vi "DiffDrivePoseEst2_AddVisionMeasurement.vi"(9 "TImeStamp_Seconds":dbl=0.02, 10 "visionRobotPose":T6={"TRANSLATION"={"X"=0.0, "Y"=0.0}, "ROTATION"={"VALUE"=0.0, "COS"=1.0, "SIN"=0.0}} {"ROTATION"."SIN" format="%13.4f"; "ROTATION"."COS" format="%13.4f"; "ROTATION"."VALUE" format="%13.4f"; "TRANSLATION"."Y" format="%14.3f"; "TRANSLATION"."X" format="%14.3f"}, 11 "in DiffDrivePoseEst2":T1={"M_Vision_K"=[], "m_nominal_dT"=0.0, "m_PrevTime_Sec"=0.0, "Pose_Buffer"={"TimeStamps"=[], "DataArray"=[], "Min_TimeStamp"=0.0, "Max_TimeStamp"=0.0, "ItemCount"=0, "MaxBufferTime"=0.0}, "Diff_Drive_Kinematics"={"TrackWidth_Meters"=0.0}, "Diff_Drive_Odom_2"={"M_POSE_Meters"={"TRANSLATION"={"X"=0.0, "Y"=0.0}, "ROTATION"={"VALUE"=0.0, "COS"=1.0, "SIN"=0.0}}, "M_GyroOffset"={"VALUE"=0.0, "COS"=1.0, "SIN"=0.0}, "M_PrevAngle"={"VALUE"=0.0, "COS"=1.0, "SIN"=0.0}, "M_PrevLeftDist_M"=0.0, "M_PrevRightDist_M"=0.0, "M_InitLeftDist_M"=0.0, "M_InitRightDist_M"=0.0}, "M_Q"=[[0.0], [0.0], [0.0]]} {"Diff_Drive_Odom_2"."M_PrevAngle"."SIN" format="%13.4f"; "Diff_Drive_Odom_2"."M_PrevAngle"."COS" format="%13.4f"; "Diff_Drive_Odom_2"."M_PrevAngle"."VALUE" format="%13.4f"; "Diff_Drive_Odom_2"."M_GyroOffset"."SIN" format="%13.4f"; "Diff_Drive_Odom_2"."M_GyroOffset"."COS" format="%13.4f"; "Diff_Drive_Odom_2"."M_GyroOffset"."VALUE" format="%13.4f"; "Diff_Drive_Odom_2"."M_POSE_Meters"."ROTATION"."SIN" format="%13.4f"; "Diff_Drive_Odom_2"."M_POSE_Meters"."ROTATION"."COS" format="%13.4f"; "Diff_Drive_Odom_2"."M_POSE_Meters"."ROTATION"."VALUE" format="%13.4f"; "Diff_Drive_Odom_2"."M_POSE_Meters"."TRANSLATION"."Y" format="%14.3f"; "Diff_Drive_Odom_2"."M_POSE_Meters"."TRANSLATION"."X" format="%14.3f"; "Diff_Drive_Kinematics"."TrackWidth_Meters" format="%20.4f"}) -> (0 "Error":bool, 3 "Out DiffDrivePoseEst2":T1={"M_Vision_K"=[], "m_nominal_dT"=0.0, "m_PrevTime_Sec"=0.0, "Pose_Buffer"={"TimeStamps"=[], "DataArray"=[], "Min_TimeStamp"=0.0, "Max_TimeStamp"=0.0, "ItemCount"=0, "MaxBufferTime"=0.0}, "Diff_Drive_Kinematics"={"TrackWidth_Meters"=0.0}, "Diff_Drive_Odom_2"={"M_POSE_Meters"={"TRANSLATION"={"X"=0.0, "Y"=0.0}, "ROTATION"={"VALUE"=0.0, "COS"=1.0, "SIN"=0.0}}, "M_GyroOffset"={"VALUE"=0.0, "COS"=1.0, "SIN"=0.0}, "M_PrevAngle"={"VALUE"=0.0, "COS"=1.0, "SIN"=0.0}, "M_PrevLeftDist_M"=0.0, "M_PrevRightDist_M"=0.0, "M_InitLeftDist_M"=0.0, "M_InitRightDist_M"=0.0}, "M_Q"=[[0.0], [0.0], [0.0]]} {"Diff_Drive_Odom_2"."M_PrevAngle"."SIN" format="%13.4f"; "Diff_Drive_Odom_2"."M_PrevAngle"."COS" format="%13.4f"; "Diff_Drive_Odom_2"."M_PrevAngle"."VALUE" format="%13.4f"; "Diff_Drive_Odom_2"."M_GyroOffset"."SIN" format="%13.4f"; "Diff_Drive_Odom_2"."M_GyroOffset"."COS" format="%13.4f"; "Diff_Drive_Odom_2"."M_GyroOffset"."VALUE" format="%13.4f"; "Diff_Drive_Odom_2"."M_POSE_Meters"."ROTATION"."SIN" format="%13.4f"; "Diff_Drive_Odom_2"."M_POSE_Meters"."ROTATION"."COS" format="%13.4f"; "Diff_Drive_Odom_2"."M_POSE_Meters"."ROTATION"."VALUE" format="%13.4f"; "Diff_Drive_Odom_2"."M_POSE_Meters"."TRANSLATION"."Y" format="%14.3f"; "Diff_Drive_Odom_2"."M_POSE_Meters"."TRANSLATION"."X" format="%14.3f"; "Diff_Drive_Kinematics"."TrackWidth_Meters" format="%20.4f"})   [LabVIEW 2019, in "Trajectory_Library.lvlib"]
doc: "Add a vision measurement to the Unscented Kalman Filter. This will correct the odometry pose estimate while still accounting for measurement noise.\n \nThis method can be called as infrequently as you want, as long as you are calling DifferentialDrivePoseEstimator_update every loop.\n\nTo promote stability of the pose estimate and make it robust to bad vision data, we recommend only adding vision measurements that are already within one meter or so of the current pose estimate.\n\n Inputs:\n - InDIffDrivePoseEstimate -- Data cluster for this system\n - visionRobotPoseMeters -- The pose of the robot as measured by the vision camera.\n - timestampSeconds -- The timestamp of the vision measurement in seconds. Note that if you don't use your own time source by calling DifferentialDrivePoseEstimator_updateWithTime then you must use a timestamp with an epoch since FPGA startup (i.e. the epoch of this timestamp is the same epoch as Timer.getFPGATimestamp.) This means that you should use Timer.getFPGATimestamp as your time source in this case.\n\nOutputs:\n - OutDIffDrivePoseEstimate -- Data cluster for this system\n - Error -- Returns TRUE if an error occured."
uses:
  Trajectory_Library.lvlib
  TypeDef/DIFF_DRIVE_POSE_EST2.ctl
  <vilib>/Analysis/Matrix/Datatypes/RealMatrix.ctl
  TypeDef/TIME_INTERPOLATABLE_VARIANT.ctl
  TypeDef/DIFF_DRIVE_KINEMATICS.ctl
  TypeDef/DIFF_DRIVE_ODOM2.ctl
  TypeDef/POSE2D.ctl
  TypeDef/TRANSLATION2D.ctl
  TypeDef/ROTATION2D.ctl
  <vilib>/Analysis/baseanly.llb/Real A x B.vi
  MatBuilder_Create.vi
  Pose2d_getRotation.vi
  Rotation2d_Minus.vi
  TimeInterpVariant_CleanUp.vi
  Rotation2d_UnaryMinus.vi
  Rotation2d_RotateBy.vi
  Rotation2d_CreateAngle.vi
  Rotation2d_CreateXY.vi
  Util_CalcDist.vi
  <vilib>/gmath/interp.llb/Search Ordered Table.vi
  DiffDrivePoseEst2_InterpRecord_Interp.vi
  <vilib>/Analysis/NI_AALBase.lvlib
  <vilib>/Analysis/Matrix/NI_Matrix.lvlib
panel:
  # "NOT A PARAMETER, JUST A DATA TYPE"
  # "<3, 1>"
  # "<3, 3>"
  # "<3, 1>"
  # "<3, 3>"
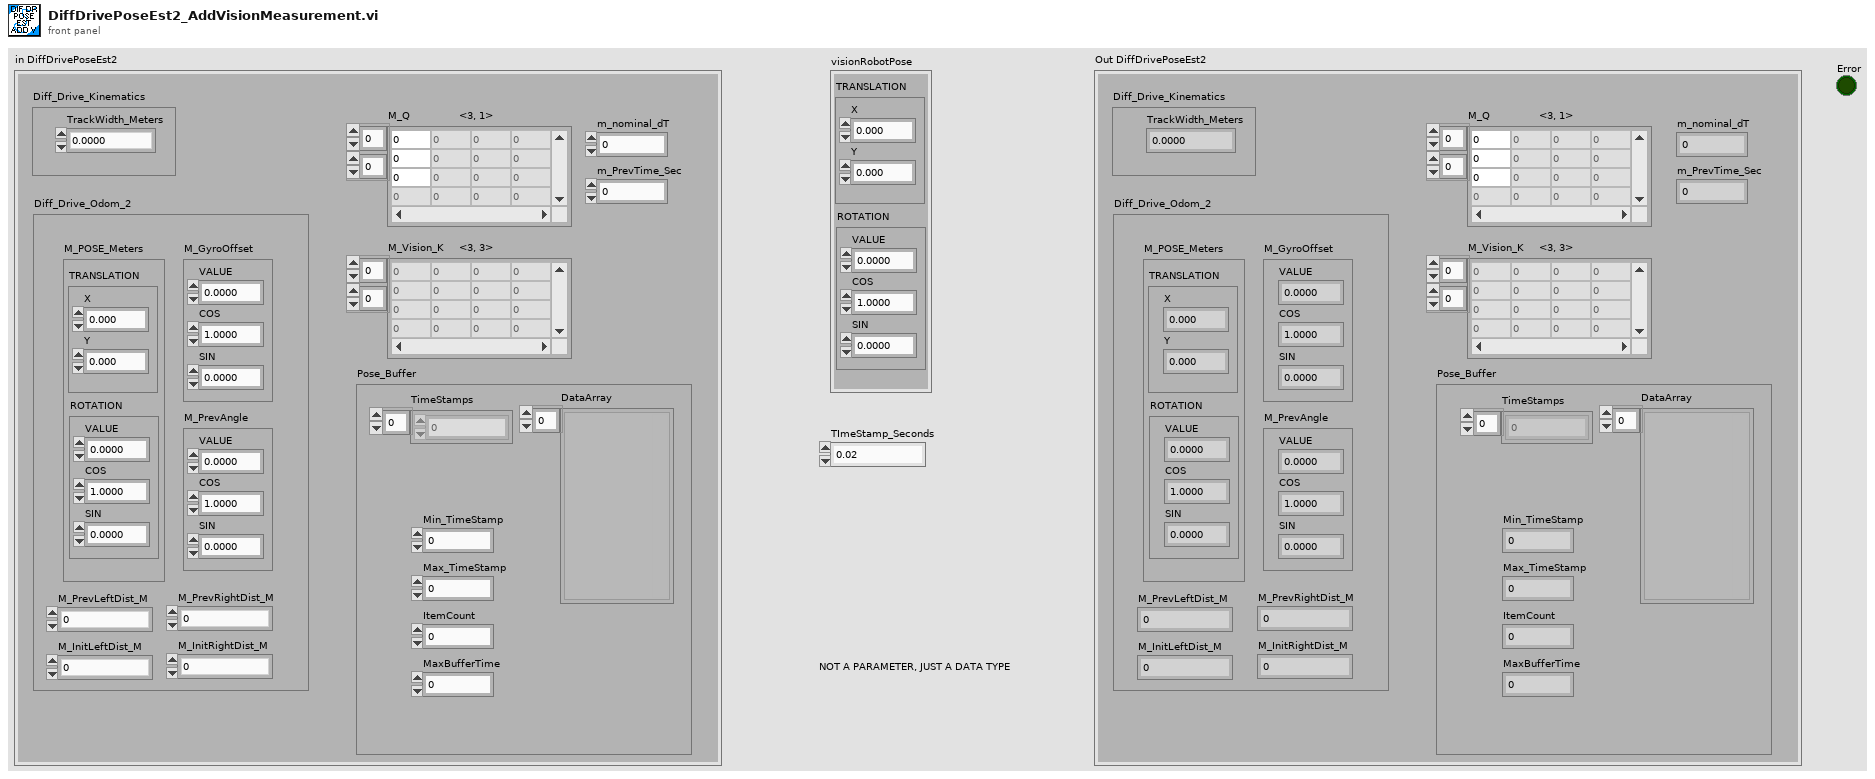
[diagram p1: front panel]
types:
  T1 = typedef "Trajectory_Library.lvlib/DIFF_DRIVE_POSE_EST2.ctl" = cluster{"M_Vision_K":T2, "m_nominal_dT":dbl, "m_PrevTime_Sec":dbl, "Pose_Buffer":T3, "Diff_Drive_Kinematics":T4, "Diff_Drive_Odom_2":T5, "M_Q":T2}
  T2 = typedef "NI_Matrix.lvlib/RealMatrix.ctl" = dbl[][]
  T3 = typedef "Trajectory_Library.lvlib/TIME_INTERPOLATABLE_VARIANT.ctl" = cluster{"TimeStamps":dbl[], "DataArray":variant[], "Min_TimeStamp":dbl, "Max_TimeStamp":dbl, "ItemCount":i32, "MaxBufferTime":dbl}
  T4 = typedef "Trajectory_Library.lvlib/DIFF_DRIVE_KINEMATICS.ctl" = cluster{"TrackWidth_Meters":dbl}
  T5 = typedef "Trajectory_Library.lvlib/DIFF_DRIVE_ODOM2.ctl" = cluster{"M_POSE_Meters":T6, "M_GyroOffset":T8, "M_PrevAngle":T8, "M_PrevLeftDist_M":dbl, "M_PrevRightDist_M":dbl, "M_InitLeftDist_M":dbl, "M_InitRightDist_M":dbl}
  T6 = typedef "Trajectory_Library.lvlib/POSE2D.ctl" = cluster{"TRANSLATION":T7, "ROTATION":T8}
  T7 = typedef "Trajectory_Library.lvlib/TRANSLATION2D.ctl" = cluster{"X":dbl, "Y":dbl}
  T8 = typedef "Trajectory_Library.lvlib/ROTATION2D.ctl" = cluster{"VALUE":dbl, "COS":dbl, "SIN":dbl}
  T9 = typedef "Trajectory_Library.lvlib/DIFF_DRIVE_POSE_EST2_INTERP_RECORD.ctl" = cluster{"PoseMeters":T6, "GyroAngle":T8, "LeftMeters":dbl, "RightMeters":dbl}
  T10 = typedef "Trajectory_Library.lvlib/TWIST2D.ctl" = cluster{"dX":dbl, "dY":dbl, "dTHETA":dbl}
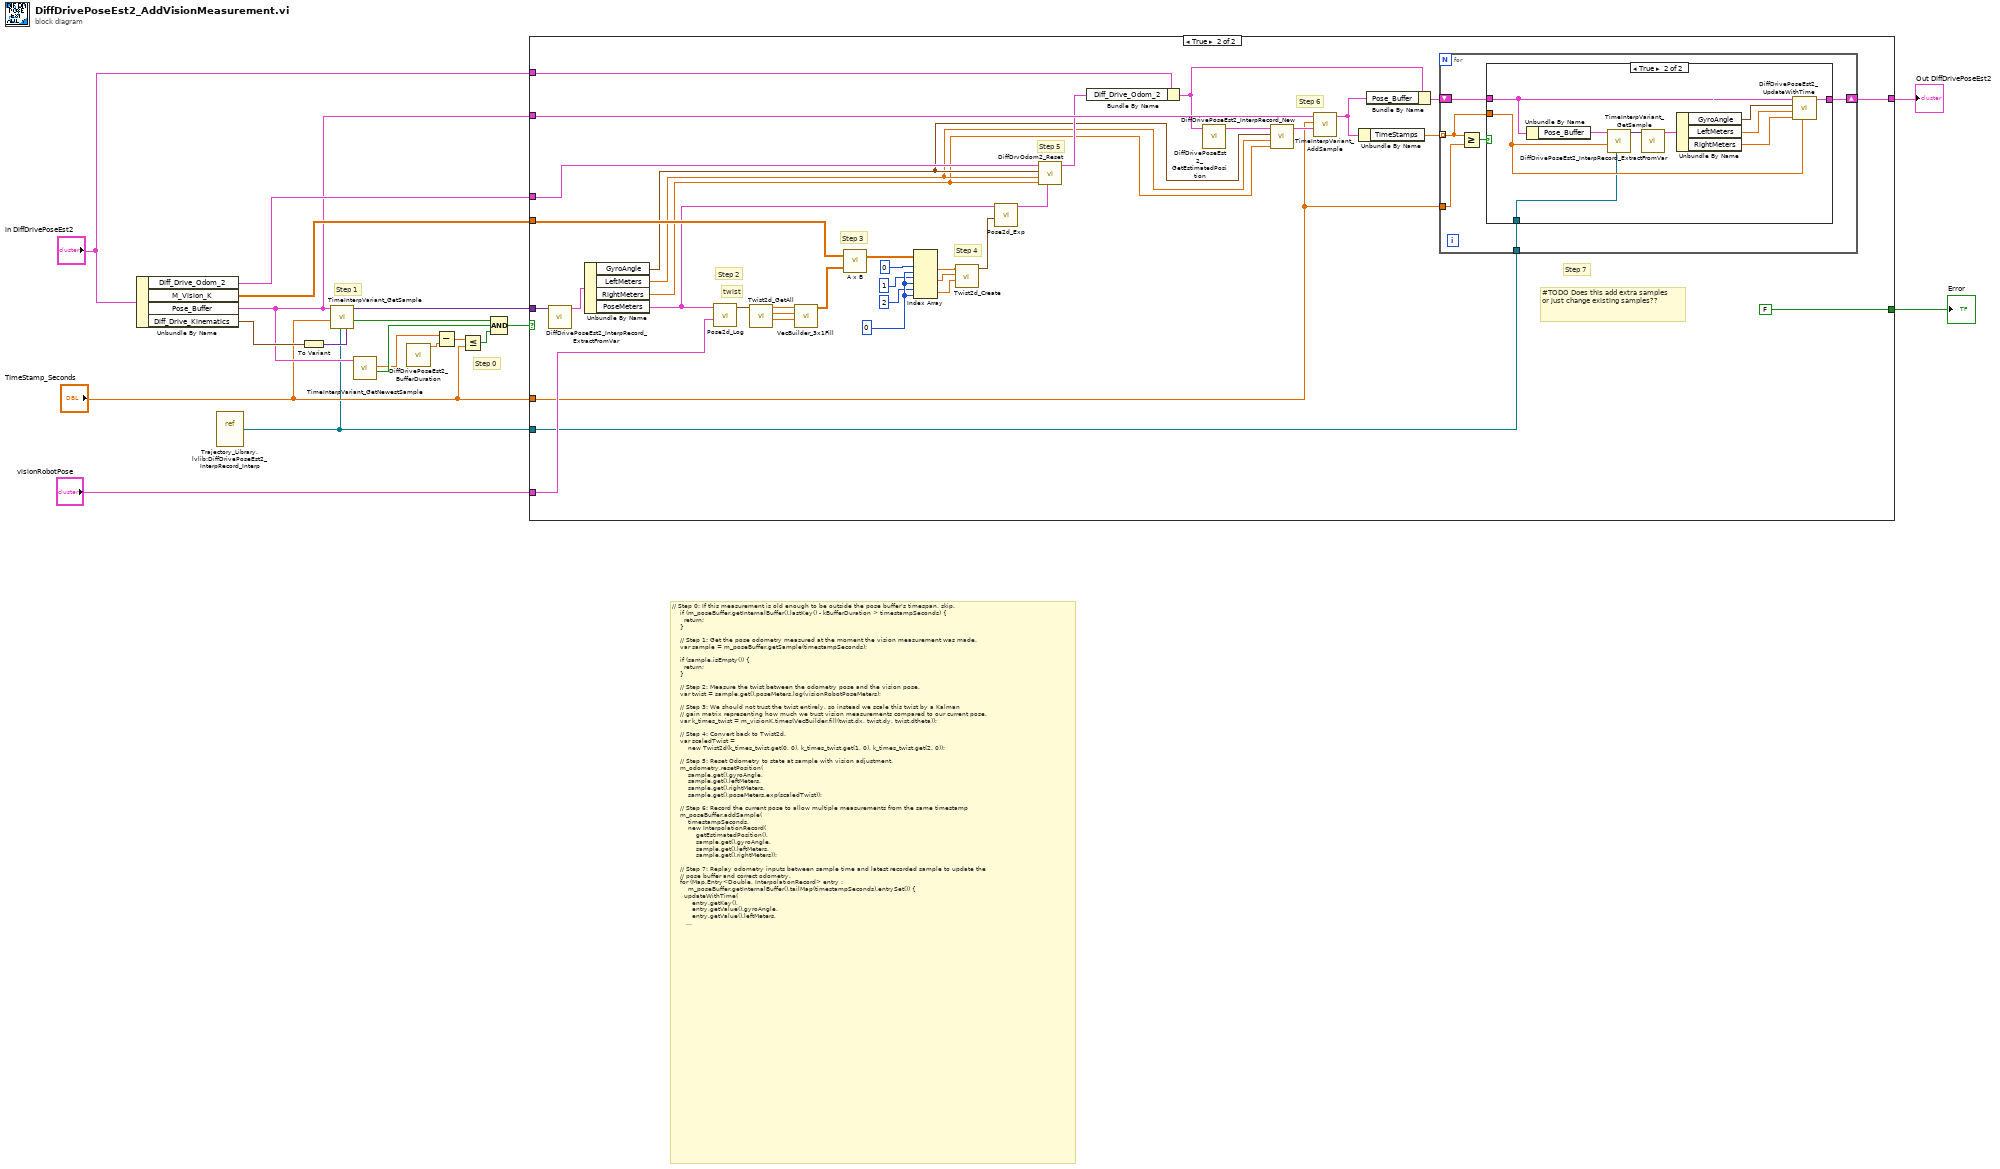
[diagram p0: block diagram]
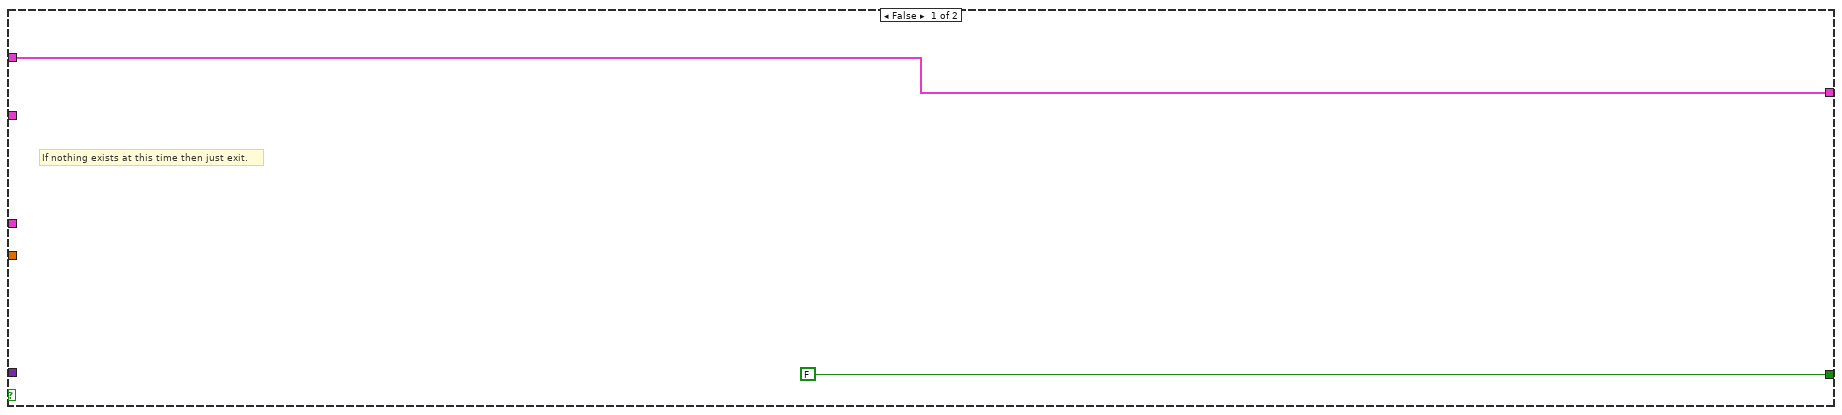
[diagram p2: hidden frame]
diagram:
  # "Step 0"
  # "Step 1"
  # "// Step 0: If this measurement is old enough to be outside the pose buffer's timespan, skip.\n    if (m_poseBuffer.getInternalBuffer().lastKey() - kBufferDuration > timestampSeconds) {\n      return;\n    }\n\n    // Step 1: Get the pose odometry measured at the moment the vision measurement was made.\n    var sample = m_poseBuffer.getSample(timestampSeconds);\n\n    if (sample.isEmpty()) {\n      return;\n    }\n\n    // Step 2: Measure the twist between the odometry pose and the vision pose.\n    var twist = sample.get().poseMeters.log(visionRobotPoseMeters);\n\n    // Step 3: We should not trust the twist entirely, so instead we scale this twist by a Kalman\n    // gain matrix representing how much we trust vision measurements compared to our current pose.\n    var k_times_twist = m_visionK.times(VecBuilder.fill(twist.dx, twist.dy, twist.dtheta));\n\n    // Step 4: Convert back to Twist2d.\n    var scaledTwist =\n        new Twist2d(k_times_twist.get(0, 0), k_times_twist.get(1, 0), k_times_twist.get(2, 0));\n\n    // Step 5: Reset Odometry to state at sample with vision adjustment.\n    m_odometry.resetPosition(\n        sample.get().gyroAngle,\n        sample.get().leftMeters,\n        sample.get().rightMeters,\n        sample.get().poseMeters.exp(scaledTwist));\n\n    // Step 6: Record the current pose to allow multiple measurements from the same timestamp\n    m_poseBuffer.addSample(\n        timestampSeconds,\n        new InterpolationRecord(\n            getEstimatedPosition(),\n            sample.get().gyroAngle,\n            sample.get().leftMeters,\n            sample.get().rightMeters));\n\n    // Step 7: Replay odometry inputs between sample time and latest recorded sample to update the\n    // pose buffer and correct odometry.\n    for (Map.Entry<Double, InterpolationRecord> entry :\n        m_poseBuffer.getInternalBuffer().tailMap(timestampSeconds).entrySet()) {\n      updateWithTime(\n          entry.getKey(),\n          entry.getValue().gyroAngle,\n          entry.getValue().leftMeters,\n          entry.getValue().rightMeters);\n    }"
  n1 = Unbundle By Name("in DiffDrivePoseEst2") -> ("Diff_Drive_Odom_2"=w11:T5, "M_Vision_K"=w12:T2, "Pose_Buffer"=w10:T3, "Diff_Drive_Kinematics"=w14:T4)
  n2 = vi-ref "Trajectory_Library.lvlib:DiffDrivePoseEst2_InterpRecord_Interp.vi"() -> (w1:refnum<vi>)
  n3 = To Variant(anything=w14) -> (Variant=w15:variant)
  n4 = call "TimeInterpVariant_GetSample.vi"("Extra"=w15, "Interpolate\nReference"=w1, "TimeStamp"="TImeStamp_Seconds", "TimeInterpVariant"=w10) -> ("IsPresent"=w9:bool, "OutputVariant"=w13:variant)  [unwired: 6 in]
  n5 = call "TimeInterpVariant_GetNewestSample.vi"("TimeInterpVariant"=w10) -> ("IsPresent"=w8:bool, "TimeStamp"=w7:dbl)  [unwired: 8 in, 1 out]
  n6 = call "DiffDrivePoseEst2_BufferDuration.vi"() -> ("Buffer Duration (Sec)"=w3:dbl)  [unwired: 11 in]
  n7 = Subtract(x=w7, y=w3) -> (x-y=w6:dbl)
  n8 = Less Or Equal?(x=w6, y="TImeStamp_Seconds") -> (x <= y?=w5:bool)
  n9 = Compound Arithmetic op=AND(w9, w8, w5) -> (w4:bool)
  n10 = case shown="True" w4 {
    tunnel: [w21 w24] -> w19
    tunnel: "visionRobotPose" -> [_ w56]
    tunnel: [FALSE FALSE] -> w17
    tunnel: "in DiffDrivePoseEst2" -> [w21 w35]
    tunnel: w13 -> [_ w58]
    tunnel: w12 -> [_ w55]
    tunnel: w11 -> [_ w41]
    tunnel: w10 -> [_ w37]
    tunnel: "TImeStamp_Seconds" -> [_ w28]
    tunnel: w1 -> [_ w22]
    frame False {
      # "If nothing exists at this time then just exit."
    }
    frame True {
      w48 = 0 ("index (col)")
      # "#TODO Does this add extra samples\nor just change existing samples??"
      # "Step 7"
      # "Step 6"
      # "Step 5"
      # "Step 4"
      # "Step 3"
      # "twist"
      # "Step 2"
      n11 = call "DiffDrivePoseEst2_InterpRecord_ExtractFromVar.vi"("OutputVariant"=w58) -> ("out InterpRecord"=w57:T9)  [unwired: 9 in, 1 out]
      n12 = Unbundle By Name(w57) -> ("GyroAngle"=w32:T8, "LeftMeters"=w31:dbl, "RightMeters"=w30:dbl, "PoseMeters"=w40:T6)
      n13 = call "Pose2d_Log.vi"("end POSE"=w56, "in POSE"=w40) -> ("out TWIST"=w54:T10)  [unwired: 9 in]
      n14 = call "Twist2d_GetAll.vi"("TWIST"=w54) -> ("dTHETA"=w51:dbl, "dY"=w52:dbl, "dX"=w53:dbl)  [unwired: 8 in]
      n15 = call "VecBuilder_3x1Fill.vi"("R2"=w51, "R1"=w52, "R0"=w53) -> ("output matrix"=w50:T2)  [unwired: 8 in]
      n16 = call-poly <vilib>:"A x B.vi"("B"=w50, "A"=w55) -> ("A x B"=w49:T2)  [unwired: 1 out]
      n17 = Index Array(array=w49, index (row) #1=0 ("index (row)"), index (col) #1=w48, index (row) #2=1 ("index (row)"), index (col) #2=w48, index (row) #3=2 ("index (row)"), index (col) #3=w48) -> (element #1=w44:dbl, element #2=w43:dbl, element #3=w42:dbl)
      n18 = call "Twist2d_Create.vi"("dTHETA"=w42, "dY"=w43, "dX"=w44) -> ("TWIST"=w39:T10)  [unwired: 8 in]
      n19 = call "Pose2d_Exp.vi"("TWIST"=w39, "POSE"=w40) -> ("UpdatedPose"=w38:T6)  [unwired: 9 in]
      n20 = call "DiffDrvOdom2_Reset.vi"("Pose Meters"=w38, "Right Distance M"=w30, "Left Distance M"=w31, "Gyro Reading"=w32, "In DIFF_DRIVE_ODOM"=w41) -> ("Out DIFF_DRIVE_ODOM"=w34:T5)  [unwired: 6 in]
      n21 = Bundle By Name(cluster=w35, "Diff_Drive_Odom_2"=w34) -> (w27:T1)
      n22 = call "DiffDrivePoseEst2_GetEstimatedPosition.vi"("in DiffDrivePoseEstimate"=w27) -> ("Estimated Pose"=w33:T6)  [unwired: 10 in]
      n23 = call "DiffDrivePoseEst2_InterpRecord_New.vi"("RightDistance"=w30, "LeftDistance"=w31, "GyroAngle"=w32, "M_POSE_Meters"=w33) -> ("DIFF_DRIVE_POSE_EST2_INTERP_RECORD"=w36:T9)  [unwired: 7 in]
      n24 = call "TimeInterpVariant_AddSample.vi"("Variant"=w36, "TimeStamp"=w28, "in TimeInterpVariant"=w37) -> ("out TimeInterpVariant"=w26:T3)  [unwired: 7 in, 1 out]
      n25 = Unbundle By Name(w26) -> ("TimeStamps"=w29:dbl[])
      n26 = Bundle By Name(cluster=w27, "Pose_Buffer"=w26) -> (w25:T1)
      n27 = for {
        tunnel: w29 -> [w63] mode=indexing
        tunnel: w28 -> [w60]
        shift-right: [w61] -> w24
        shift-left: w25 -> [w62]
        tunnel: w22 -> [w59]
        n28 = Greater Or Equal?(x=w63, y=w60) -> (x >= y?=w64:bool)
        n29 = case shown="True" w64 {
          tunnel: w63 -> [_ w67]
          tunnel: w62 -> [w65 w70]
          tunnel: [w65 w75] -> w61
          tunnel: w59 -> [_ w66]
          frame False {
          }
          frame True {
            n30 = Unbundle By Name(w70) -> ("Pose_Buffer"=w69:T3)
            n31 = call "TimeInterpVariant_GetSample.vi"("Extra"=w67, "Interpolate\nReference"=w66, "TimeStamp"=w67, "TimeInterpVariant"=w69) -> ("OutputVariant"=w68:variant)  [unwired: 6 in, 1 out]
            n32 = call "DiffDrivePoseEst2_InterpRecord_ExtractFromVar.vi"("OutputVariant"=w68) -> ("out InterpRecord"=w74:T9)  [unwired: 9 in, 1 out]
            n33 = Unbundle By Name(w74) -> ("GyroAngle"=w73:T8, "LeftMeters"=w72:dbl, "RightMeters"=w71:dbl)
            n34 = call "DiffDrivePoseEst2_UpdateWithTime.vi"("CurrentTimeSeconds"=w67, "RightDistance"=w71, "LeftDistance"=w72, "GyroAngle"=w73, "in DiffDrivePoseEst2"=w70) -> ("Out DiffDrivePoseEst2"=w75:T1)  [unwired: 4 in, 2 out]
          }
        }
      }
    }
  }
  "Out DiffDrivePoseEst2" <- w19
  "Error" <- w17
